vi "lvmcp_concat.vi"() -> ()   [LabVIEW 2015]
panel:
  out "error out":errorcluster
  in  "concatenate":bool
  in  "reference":refnum<vi>
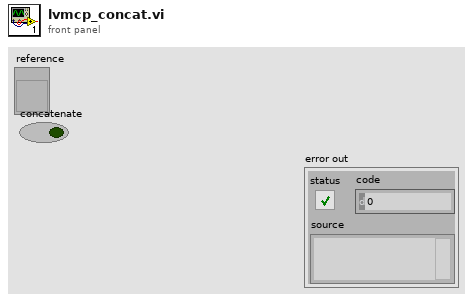
[diagram p1: front panel]
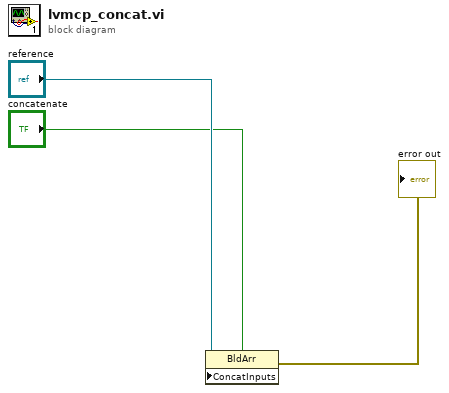
[diagram p0: block diagram]
diagram:
  n1 = property class="BldArr"(reference="reference", "ConcatInputs"="concatenate") -> (error out=→"error out":errorcluster)  [unwired: 1 in, 1 out]
